vi "sandbox flatten unflatten.vi"() -> ()   [LabVIEW 2019, in "XPUB.lvclass"]
uses:
  XPUB.lvclass
  <vilib>/LabVIEW Open Source Project/Epoch Date & Time/formatter.iso8601/Seconds Units -- enum.ctl
  <vilib>/numeric/Random Number (Range) DBL.vi
  <vilib>/ptbypt/NI_PtbyPt.lvlib
panel:
  out "sum prepare + flatten":dbl format="%#_6p"
  in  "stop":bool
  out "output cluster":T1
  out "x = y?":bool
  out "unflatten":dbl format="%#_6p"
  out "manipulate unflattened":dbl format="%#_6p"
  out "prepare for flatten":dbl format="%#_6p"
  out "flatten":dbl format="%#_6p"
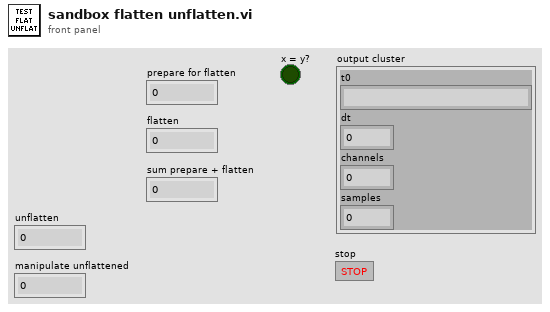
[diagram p1: front panel]
types:
  T1 = cluster{"t0":string, "dt":dbl, "channels":i32, "samples":i32}
  T2 = typedef "Seconds Units -- enum.ctl" = enum16{"second", "millisecond", "microsecond", "nanosecond"}
  T3 = enum16{"big-endian, network order", "native, host order", "little-endian"}
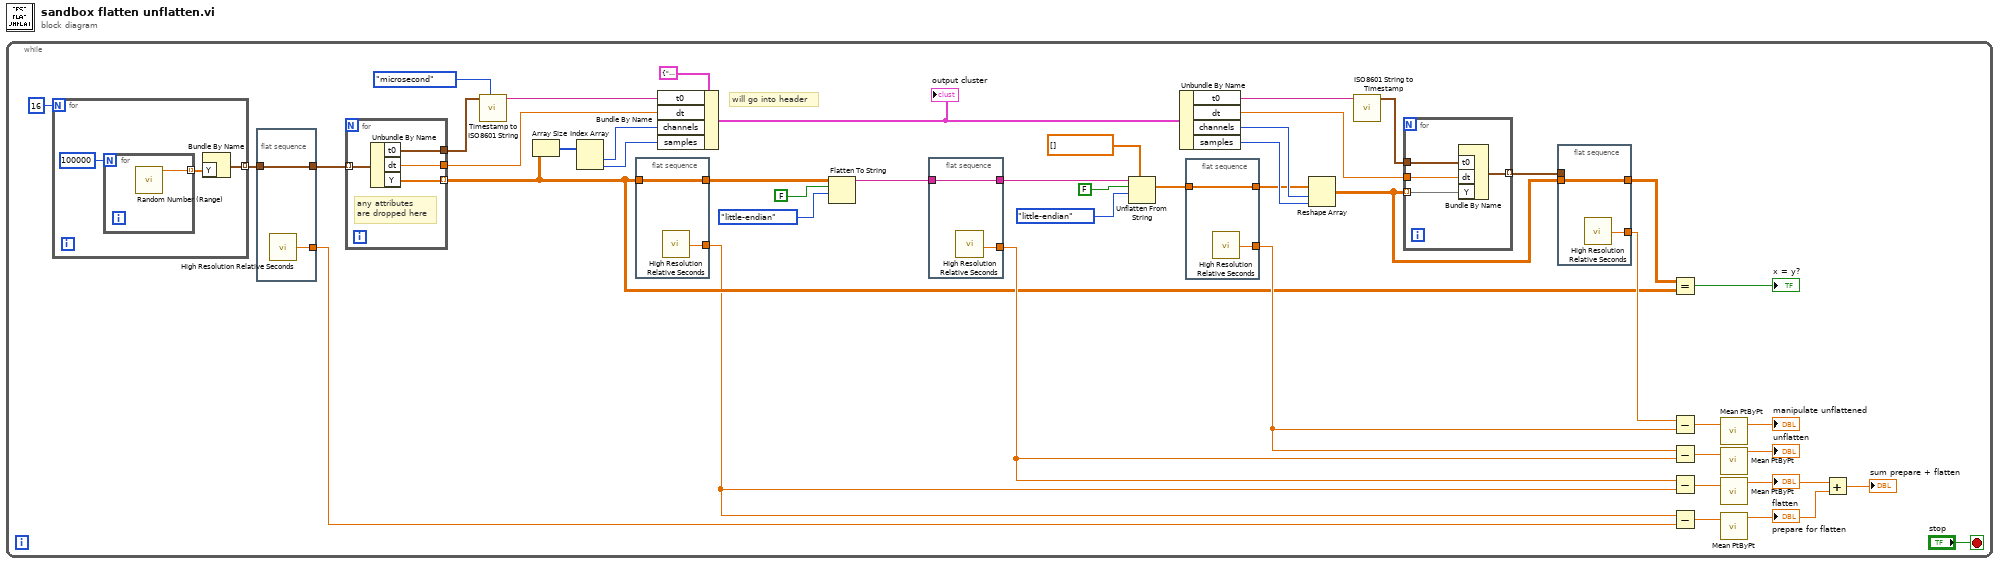
[diagram p0: block diagram]
diagram:
  n1 = while {
    stop <- "stop" stop-if-true
    # "will go into header"
    n2 = for {
      N: 16 -> [_]
      tunnel: [w63] -> w35 mode=indexing
      n3 = for {
        N: 100000 -> [_]
        tunnel: [w65] -> w64 mode=indexing
        n4 = call-poly <vilib>:"Random Number (Range).vi"() -> ("number"=w65:dbl)  [unwired: 11 in]
      }
      n5 = Bundle By Name("Y"=w64) -> (w63:waveform(dbl))  [unwired: 1 in]
    }
    n6 = flat-sequence {
      tunnel: w35 -> [w57]
      tunnel: [w57] -> w16
      tunnel: [w56] -> w14
      frame #0 {
        n7 = call <vilib>:"High Resolution Relative Seconds.vi"() -> ("relative seconds"=w56:dbl)
      }
    }
    n8 = for {
      tunnel: w16 -> [w58] mode=indexing
      tunnel: [w61] -> w4 mode=indexing
      tunnel: [w60] -> w23
      tunnel: [w59] -> w12
      # "any attributes\nare dropped here"
      n9 = Unbundle By Name(w58) -> ("t0"=w60:timestamp, "dt"=w59:dbl, "Y"=w61:dbl[])
    }
    n10 = call <vilib>:"Timestamp to ISO8601 String.vi"("Unit (ms)"=Seconds_Units_--_enum."microsecond", "Timestamp (now)"=w23) -> ("ISO8601 String"=w22:string)  [unwired: 9 in]
    n11 = Array Size(array=w4) -> (size(s)=w42:i32[])
    n12 = Index Array(array=w42) -> (element #1=w41:i32, element #2=w40:i32)  [unwired: 2 in]
    n13 = flat-sequence {
      tunnel: w4 -> [w55]
      tunnel: [w55] -> w34
      tunnel: [w54] -> w2
      frame #0 {
        n14 = call <vilib>:"High Resolution Relative Seconds.vi"() -> ("relative seconds"=w54:dbl)
      }
    }
    n15 = Bundle By Name(cluster=T1 {"t0"="", "dt"=0.0, "channels"=0, "samples"=0}, "t0"=w22, "dt"=w12, "channels"=w41, "samples"=w40) -> (w39:T1)
    "output cluster" <- w39
    n16 = Flatten To String(anything=w34, prepend array or string size? (T)=FALSE, byte order (0:big-endian, network order)=T3."little-endian") -> (data string=w15:string)  [unwired: 1 in, 2 out]
    n17 = flat-sequence {
      tunnel: w15 -> [w53]
      tunnel: [w53] -> w3
      tunnel: [w52] -> w28
      frame #0 {
        n18 = call <vilib>:"High Resolution Relative Seconds.vi"() -> ("relative seconds"=w52:dbl)
      }
    }
    n19 = Unflatten From String(type=dbl[] [], binary string=w3, data includes array or string size? (T)=FALSE, byte order (0:big-endian, network order)=T3."little-endian") -> (value=w33:dbl[])  [unwired: 1 in, 2 out]
    n20 = Unbundle By Name(w39) -> ("t0"=w18:string, "dt"=w17:dbl, "channels"=w38:i32, "samples"=w37:i32)
    n21 = flat-sequence {
      tunnel: w33 -> [w51]
      tunnel: [w51] -> w31
      tunnel: [w50] -> w29
      frame #0 {
        n22 = call <vilib>:"High Resolution Relative Seconds.vi"() -> ("relative seconds"=w50:dbl)
      }
    }
    n23 = Reshape Array(w31, w38, w37) -> (w26:dbl[][])
    n24 = call <vilib>:"ISO8601 String to Timestamp.vi"("ISO8601 String"=w18) -> ("Timestamp"=w20:timestamp)  [unwired: 8 in, 2 out]
    n25 = for {
      tunnel: w26 -> [w69] mode=indexing
      tunnel: w17 -> [w68]
      tunnel: w20 -> [w67]
      tunnel: [w66] -> w25 mode=indexing
      n26 = Bundle By Name("t0"=w67, "dt"=w68, "Y"=w69) -> (w66:waveform(dbl))  [unwired: 1 in]
    }
    n27 = flat-sequence {
      tunnel: w26 -> [w49]
      tunnel: [w49] -> w32
      tunnel: [w48] -> w30
      tunnel: w25 -> [_]
      frame #0 {
        n28 = call <vilib>:"High Resolution Relative Seconds.vi"() -> ("relative seconds"=w48:dbl)
      }
    }
    n29 = Equal?(x=w32, y=w4) -> (x = y?=→"x = y?":bool)
    n30 = Subtract(x=w30, y=w29) -> (x-y=w27:dbl)
    n31 = Subtract(x=w29, y=w28) -> (x-y=w7:dbl)
    n32 = Subtract(x=w28, y=w2) -> (x-y=w8:dbl)
    n33 = Subtract(x=w2, y=w14) -> (x-y=w9:dbl)
    n34 = call <vilib>:"Mean PtByPt.vi"("x"=w27) -> ("mean"=→"manipulate unflattened":dbl)  [unwired: 3 in, 1 out]
    n35 = call <vilib>:"Mean PtByPt.vi"("x"=w7) -> ("mean"=→"unflatten":dbl)  [unwired: 3 in, 1 out]
    n36 = call <vilib>:"Mean PtByPt.vi"("x"=w8) -> ("mean"=w5:dbl)  [unwired: 3 in, 1 out]
    "flatten" <- w5
    n37 = call <vilib>:"Mean PtByPt.vi"("x"=w9) -> ("mean"=w1:dbl)  [unwired: 3 in, 1 out]
    "prepare for flatten" <- w1
    n38 = Add(x=w5, y=w1) -> (x+y=→"sum prepare + flatten":dbl)
  }
